vi "set BandWidth.vi"(8 "error in (no error)":errorcluster, 9 "LTE Channel Type":T2, 10 "BandWidth":T1, 11 "LTE in":refnum<class "LTE.lvclass">) -> (0 "error out":errorcluster, 3 "LTE out":refnum<class "LTE.lvclass">)   [LabVIEW 2023, in "ANRITSU Call Box.lvlib" / "LTE.lvclass"]
uses:
  LTE.lvclass
  Type Definition/LTE Channel Type.ctl
  Type Definition/LTE Supported BandWidth.ctl
  LTE.lvclass/LTE.ctl
  ANRITSU Call Box.lvlib
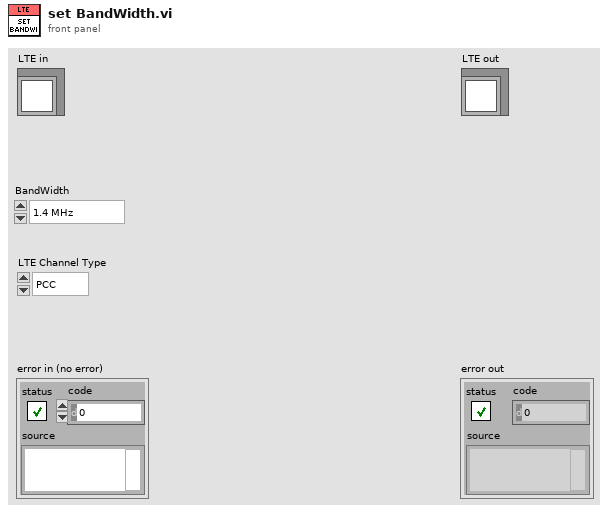
[diagram p1: front panel]
types:
  T1 = typedef "ANRITSU Call Box.lvlib/LTE Supported BandWidth.ctl" = enum16{"1.4 MHz", "3 MHz", "5 MHz", "10 MHz", "15 MHz", "20 MHz"}
  T2 = typedef "ANRITSU Call Box.lvlib/LTE Channel Type.ctl" = enum16{"PCC", "SCC1", "SCC2", "SCC3"}
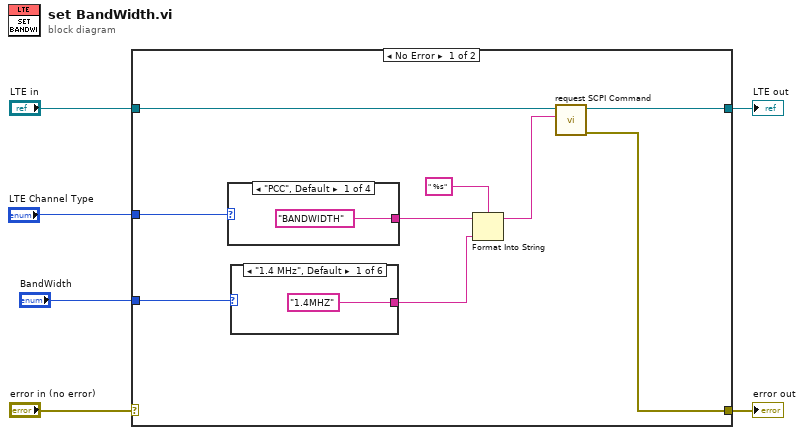
[diagram p0: block diagram]
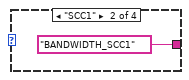
[diagram p2: hidden frame]
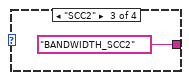
[diagram p3: hidden frame]
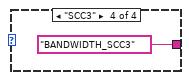
[diagram p4: hidden frame]
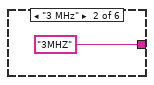
[diagram p5: hidden frame]
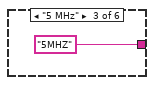
[diagram p6: hidden frame]
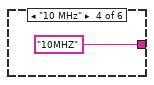
[diagram p7: hidden frame]
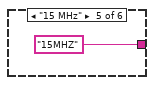
[diagram p8: hidden frame]
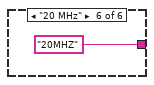
[diagram p9: hidden frame]
diagram:
  n1 = case shown="No Error" "error in (no error)" {
    selector: "error in (no error)" -> [_ w27]
    tunnel: [w8 w27] -> w5
    tunnel: [w9 w26] -> w3
    tunnel: "LTE in" -> [w7 w26]
    tunnel: "BandWidth" -> [w15 _]
    tunnel: "LTE Channel Type" -> [w14 _]
    frame No Error {
      n2 = case shown="\"PCC\", Default" w14 {
        tunnel: ["BANDWIDTH" ("string") "BANDWIDTH_SCC1" ("string") "BANDWIDTH_SCC2" ("string") "BANDWIDTH_SCC3" ("string")] -> w13
        frame "PCC", Default {
        }
        frame "SCC1" {
        }
        frame "SCC2" {
        }
        frame "SCC3" {
        }
      }
      n3 = case shown="\"1.4 MHz\", Default" w15 {
        tunnel: ["1.4MHZ" "3MHZ" "5MHZ" "10MHZ" "15MHZ" "20MHZ"] -> w11
        frame "1.4 MHz", Default {
        }
        frame "3 MHz" {
        }
        frame "5 MHz" {
        }
        frame "10 MHz" {
        }
        frame "15 MHz" {
        }
        frame "20 MHz" {
        }
      }
      n4 = Format Into String(format string=" %s", initial string=w13, w11) -> (resulting string=w10:string)  [unwired: 1 in, 1 out]
      n5 = call "request SCPI Command.vi"("SCPI Command"=w10, "LTE in"=w7) -> ("error out"=w8:errorcluster, "LTE out"=w9:refnum<class "LTE.lvclass">)  [unwired: 8 in]
    }
    frame Error {
    }
  }
  "error out" <- w5
  "LTE out" <- w3
